vi "xnet_canopen_start.vi"(8 "error in (no error)":errorcluster, 11 "xnet_co_handle_in":u64) -> (0 "error out":errorcluster, 3 "xnet_co_handle":u64)   [LabVIEW 2023, in "xnet_canopen.lvlib"]
uses:
  <vilib>/Utility/error.llb/Error Cluster From Error Code.vi
  xnet_canopen.lvlib
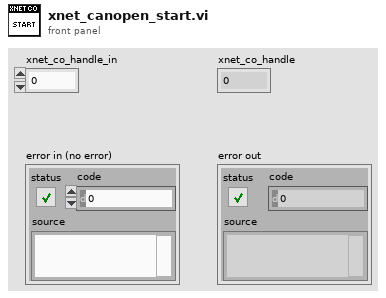
[diagram p1: front panel]
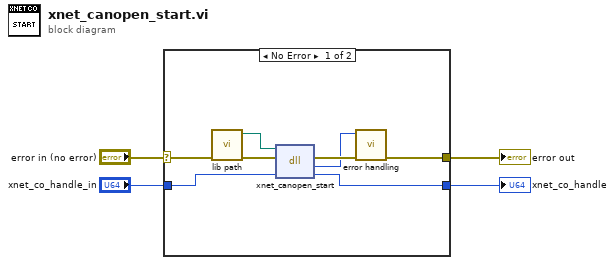
[diagram p0: block diagram]
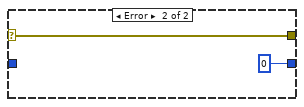
[diagram p2: hidden frame]
diagram:
  n1 = case shown="No Error" "error in (no error)" {
    selector: "error in (no error)" -> [w10 w13]
    tunnel: [w8 w13] -> w3
    tunnel: [w6 u64 0 ("phandle")] -> w2
    tunnel: "xnet_co_handle_in" -> [w5 _]
    frame No Error {
      n2 = call "lib path.vi"() -> ("lib path"=w11:path)  [unwired: 11 in]
      n3 = dll-call lib="?" fn="xnet_canopen_start"(path in=w11, error in=w10, "handle"=w5) -> (error out=w9:errorcluster, "return type"=w7:i32, "handle"=w6:u64)  [unwired: 1 in, 1 out]
      n4 = call "error handling.vi"("error in (no error)"=w9, "return val"=w7) -> ("error out"=w8:errorcluster)  [unwired: 9 in]
    }
    frame Error {
    }
  }
  "error out" <- w3
  "xnet_co_handle" <- w2
